vi "VIH ProjFile - Close.vi"(8 "error in":errorcluster, 11 "Project":T1) -> (0 "error out":errorcluster)   [LabVIEW 2014]
doc: "::: VI Helpeks :::\nCopyright (c) 2000-2026 Konstantin Shifershteyn. All rights reserved."
uses:
  <vilib>/xml/Close Reference(Node).vi
  <vilib>/xml/NI_XML.lvlib
panel:
  # "VI Helpeks\nCopyright (c) 2012-2026 Konstantin Shifershteyn"
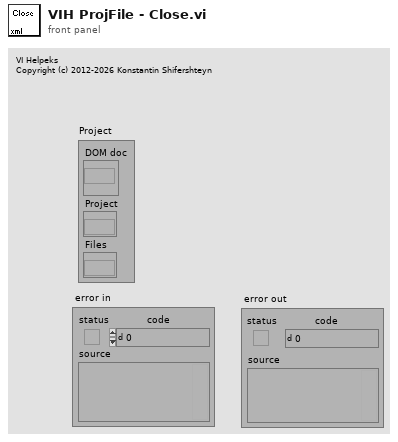
[diagram p1: front panel]
types:
  T1 = cluster{"DOM doc":refnum<k20>, "Project":refnum<k20>, "Files":refnum<k20>}
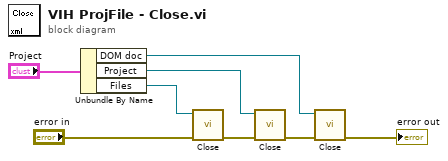
[diagram p0: block diagram]
diagram:
  n1 = Unbundle By Name("Project") -> ("DOM doc"=w2:refnum<k20>, "Project"=w3:refnum<k20>, "Files"=w4:refnum<k20>)
  n2 = call-poly <vilib>:"Close.vi"("error in (no error)"="error in", "node"=w4) -> ("error out"=w7:errorcluster)  [unwired: 7 in]
  n3 = call-poly <vilib>:"Close.vi"("error in (no error)"=w7, "node"=w3) -> ("error out"=w6:errorcluster)  [unwired: 7 in]
  n4 = call-poly <vilib>:"Close.vi"("error in (no error)"=w6, "node"=w2) -> ("error out"=→"error out":errorcluster)  [unwired: 7 in]
